vi "JUnit Simple.vi"() -> ()   [LabVIEW 2013]
doc: "This example provides a simple example for <B>JUnit XML</B>."
uses:
  JUnit XML/Test Suite/Test Suite.lvclass
  JUnit XML/Test Case/Test Case.lvclass
panel:
  out "XML":string
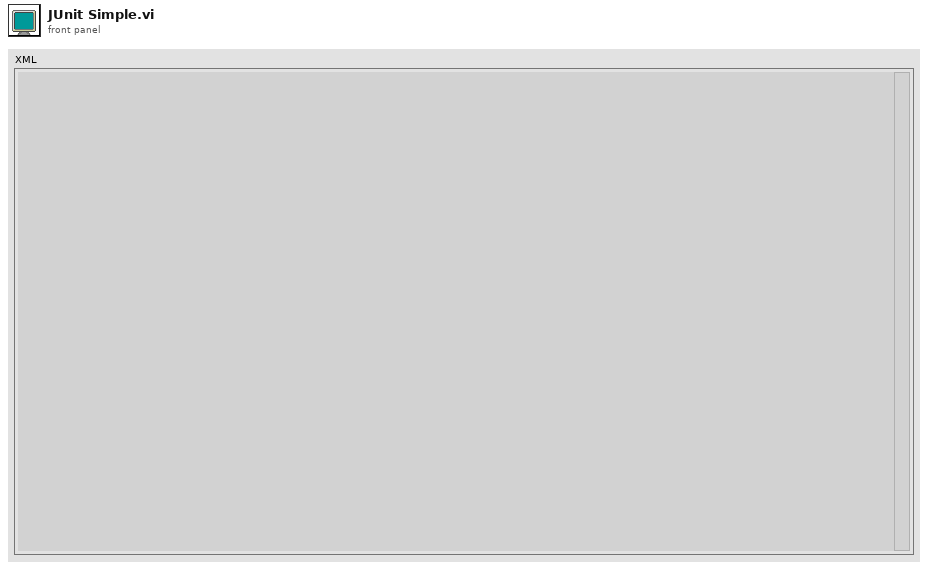
[diagram p1: front panel]
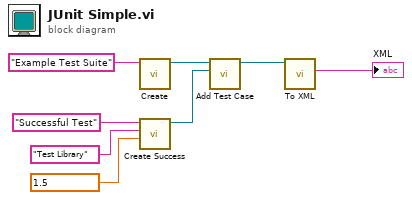
[diagram p0: block diagram]
diagram:
  n1 = call "Create.vi"("Name"="Example Test Suite") -> ("Test Suite"=w3:refnum<class "Test Suite.lvclass">)  [unwired: 9 in, 1 out]
  n2 = call "Create Success.vi"("Time"=1.5, "Classname"="Test Library", "Name"="Successful Test") -> ("Test Case"=w2:refnum<class "Test Case.lvclass">)  [unwired: 7 in, 1 out]
  n3 = call "Add Test Case.vi"("Test Case"=w2, "Test Suite in"=w3) -> ("Test Suite out"=w1:refnum<class "Test Suite.lvclass">)  [unwired: 8 in, 1 out]
  n4 = call-dynamic "To XML.vi"("Serializable in"=w1) -> ("XML"=→"XML":string)  [unwired: 9 in, 1 out]
